vi "Find Wire Segments and Distances.vi"(8 "Error":errorcluster, 9 "Co-ordinates":cluster{"x":i16, "y":i16}, 11 "Joints[]":T2(array[cluster])) -> (0 "Error Out":errorcluster, 1 "Distances":dbl[](array[numeric]), 2 "Segments":T1[](array[typedef]) {"Direction" items=["Up", "Down", "Left", "Right"]}, 3 "Terminating Joints":i32[](array[numeric]))   [LabVIEW 2012, in "Scripting Tools.lvlib"]
doc: "Given the Joints[] Property of a wire and the co-ordinates of a point, generates a list of segments and calculates the perpendicular distance of the point to each segment."
uses:
  Scripting Tools.lvlib
  Wire Segment Descriptor Type.ctl
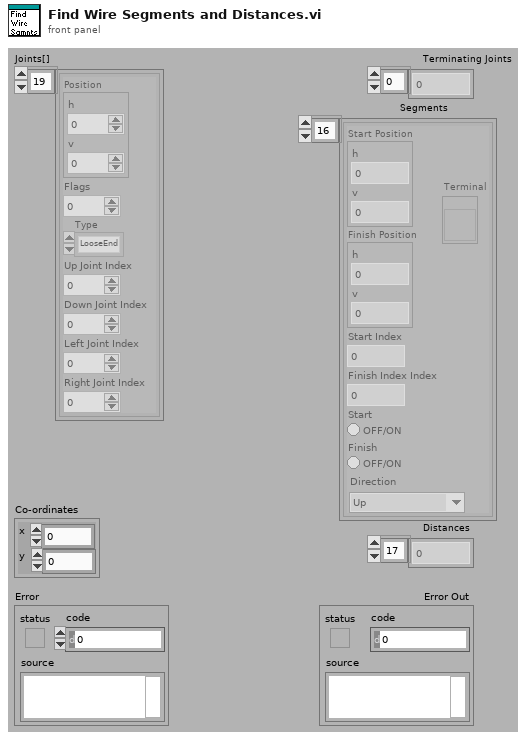
[diagram p1: front panel]
types:
  T1 = typedef "Scripting Tools.lvlib/Wire Segment Descriptor Type.ctl" = cluster{"Start Position":cluster{"h":i16, "v":i16}, "Finish Position":cluster{"h":i16, "v":i16}, "Start Index":i32, "Finish Index Index":i32, "Start":bool, "Finish":bool, "Direction":u16, "Terminal":refnum<vi>}
  T2 = cluster{"Position":cluster{"h":i16, "v":i16}, "Flags":i32, "Type":enum32{"LooseEnd", "Endpoint", "Bend", "Junction"}, "Up Joint Index":i16, "Down Joint Index":i16, "Left Joint Index":i16, "Right Joint Index":i16}[]
  T3 = enum32{"LooseEnd", "Endpoint", "Bend", "Junction"}
  T4 = cluster{"Position":cluster{"h":i16, "v":i16}, "Flags":i32, "Type":enum32{"LooseEnd", "Endpoint", "Bend", "Junction"}, "Up Joint Index":i16, "Down Joint Index":i16, "Left Joint Index":i16, "Right Joint Index":i16}
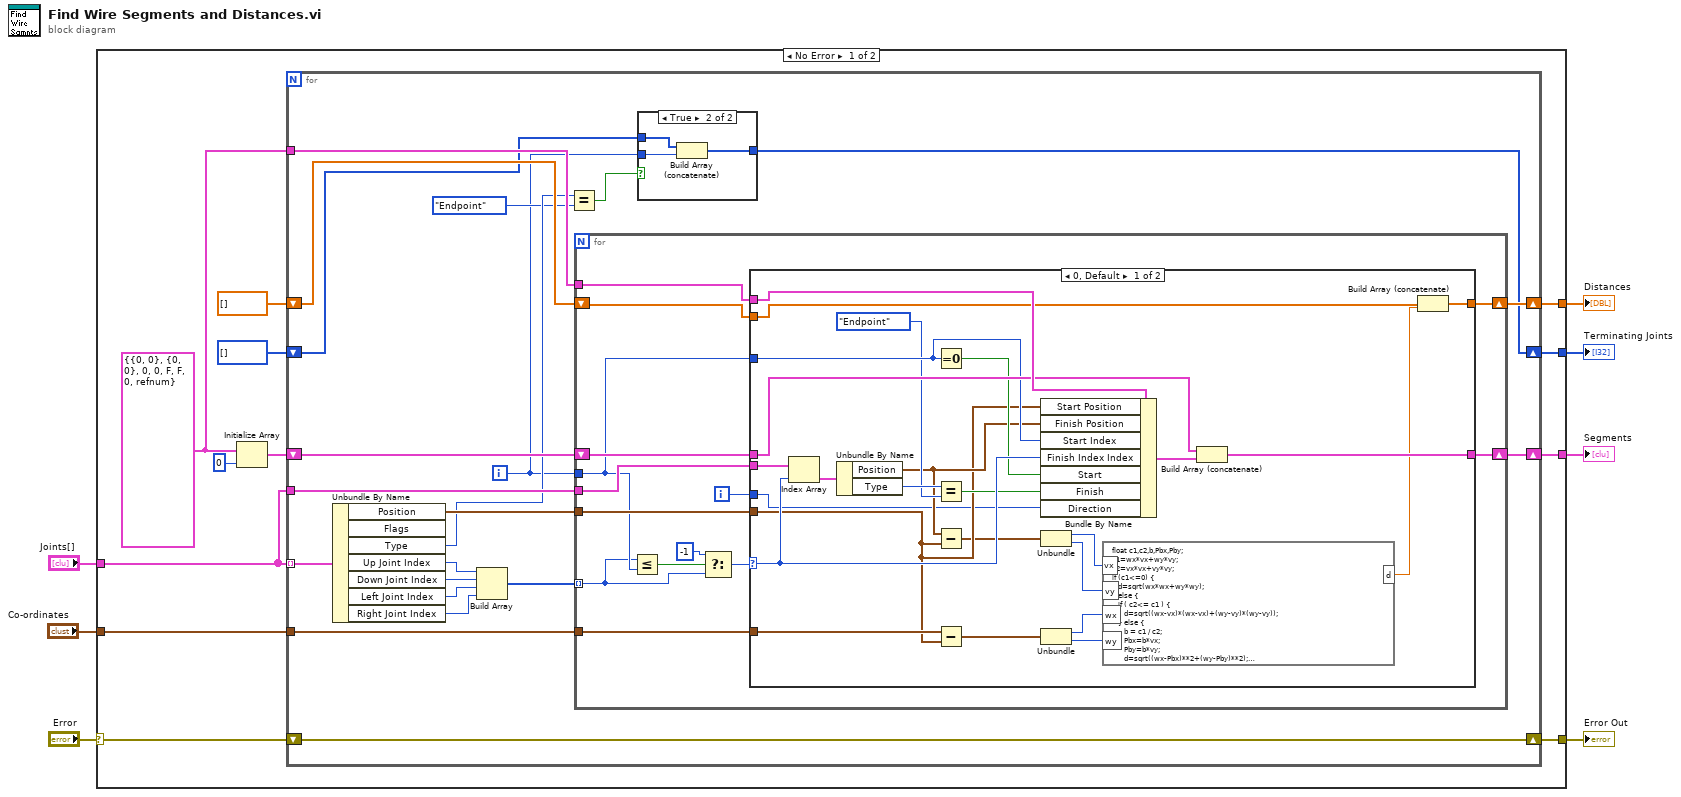
[diagram p0: block diagram]
diagram:
  n1 = case shown="No Error" "Error" {
    selector: "Error" -> [w8 w86]
    tunnel: [w19 w86] -> w7
    tunnel: "Joints[]" -> [w18 _]
    tunnel: [w17 _] -> w4
    tunnel: [w15 _] -> w3
    tunnel: [w14 _] -> w2
    tunnel: "Co-ordinates" -> [w12 _]
    frame No Error {
      w11 = T1 {"Start Position"={"h"=0, "v"=0}, "Finish Position"={"h"=0, "v"=0}, "Start Index"=0, "Finish Index Index"=0, "Start"=FALSE, "Finish"=FALSE, "Direction"=0, "Terminal"=refnum} ("Segment Descriptor")
      n2 = Initialize Array(w11, 0 ("dimension size")) -> (w10:T1[])
      n3 = for {
        tunnel: w18 -> [w40] mode=indexing
        tunnel: w18 -> [w34]
        tunnel: w11 -> [w32]
        shift-right: [w30] -> w15
        shift-left: w10 -> [w28]
        tunnel: w12 -> [w31]
        shift-right: [w29] -> w14
        shift-left: dbl[] [] -> [w27]
        shift-right: [w21] -> w17
        shift-left: i32[] [] -> [w23]
        shift-right: [w20] -> w19
        shift-left: w8 -> [w20]
        i -> [w24]
        n4 = Unbundle By Name(w40) -> ("Position"=w33:cluster{"h":i16, "v":i16}, "Type"=w26:T3, "Up Joint Index"=w39:i16, "Down Joint Index"=w38:i16, "Left Joint Index"=w37:i16, "Right Joint Index"=w36:i16)  [unwired: 1 out]
        n5 = Build Array(w39, w38, w37, w36) -> (w35:i16[])
        n6 = Equal?(x=w26, y=T3."Endpoint") -> (x = y?=w22:bool)
        n7 = for {
          tunnel: w35 -> [w47] mode=indexing
          tunnel: w34 -> [w58]
          tunnel: w33 -> [w57]
          tunnel: w32 -> [w56]
          tunnel: w24 -> [w49]
          shift-right: [w55] -> w30
          shift-left: w28 -> [w54]
          tunnel: w31 -> [w53]
          shift-right: [w52] -> w29
          shift-left: w27 -> [w51]
          i -> [w50]
          n8 = Less Or Equal?(x=w47, y=w49) -> (x <= y?=w48:bool)
          n9 = Select(t=i16 -1, s=w48, f=w47) -> (s? t:f=w46:i16)
          n10 = case shown="0, Default" w46 {
            selector: w46 -> [w81 _]
            tunnel: w58 -> [w83 _]
            tunnel: w57 -> [w70 _]
            tunnel: w56 -> [w80 _]
            tunnel: w49 -> [w76 _]
            tunnel: [w79 w85] -> w55
            tunnel: w54 -> [w78 w85]
            tunnel: w53 -> [w71 _]
            tunnel: [w62 w84] -> w52
            tunnel: w51 -> [w61 w84]
            tunnel: w50 -> [w59 _]
            frame 0, Default {
              n11 = Index Array(array=w83, index=w81) -> (element=w82:T4)
              n12 = Unbundle By Name(w82) -> ("Position"=w72:cluster{"h":i16, "v":i16}, "Type"=w74:T3)
              n13 = Equal To 0?(x=w76) -> (x = 0?=w77:bool)
              n14 = Equal?(x=w74, y=T3."Endpoint") -> (x = y?=w75:bool)
              n15 = Subtract(x=w72, y=w70) -> (x-y=w69:cluster{"h":i16, "v":i16})
              n16 = Subtract(x=w71, y=w70) -> (x-y=w68:cluster{i16, i16})
              n17 = Bundle By Name(cluster=w80, "Start Position"=w70, "Finish Position"=w72, "Start Index"=w76, "Finish Index Index"=w81, "Start"=w77, "Finish"=w75, "Direction"=w59) -> (w60:T1)
              n18 = Unbundle(w69) -> ("h"=w67:i16, "v"=w66:i16)
              n19 = Unbundle(w68) -> (w65:i16, w64:i16)
              n20 = formula code="float c1,c2,b,Pbx,Pby;\nc1=wx*vx+wy*vy;\nc2=vx*vx+vy*vy;\nif (c1<=0) {\n   d=sqrt(wx*wx+wy*wy);\n} else {\n   if ( c2<= c1 ) {\n      d=sqrt((wx-vx)*(wx-vx)+(wy-vy)*(wy-vy));\n   } else {\n      b = c1 / c2;\n      Pbx=b*vx;\n      Pby=b*vy;\n      d=sqrt((wx-Pbx)**2+(wy-Pby)**2);\n   }\n}"("vx"=w67, "vy"=w66, "wx"=w65, "wy"=w64) -> ("d"=w63:dbl)
              n21 = Build Array (concatenate)(w78, w60) -> (w79:T1[])
              n22 = Build Array (concatenate)(w61, w63) -> (w62:dbl[])
            }
            frame -1 {
            }
          }
        }
        n23 = case shown="True" w22 {
          tunnel: w24 -> [_ w44]
          tunnel: [w41 w43] -> w21
          tunnel: w23 -> [w41 w42]
          frame False {
          }
          frame True {
            n24 = Build Array (concatenate)(w42, w44) -> (w43:i32[])
          }
        }
      }
    }
    frame Error {
    }
  }
  "Error Out" <- w7
  "Terminating Joints" <- w4
  "Segments" <- w3
  "Distances" <- w2
